vi "Ctor.vi"(8 "error in (no error)":errorcluster, 10 "Role Hierarchy (None)":T1[](array[typedef])) -> (0 "error out":errorcluster, 3 "Security out":refnum<class "Security.lvclass">)   [LabVIEW 2020, in "HTTP Server.lvlib" / "Security.lvclass"]
uses:
  Security.lvclass
  Role Inheritance.ctl
  Ref Data.ctl
  Hierarchy.ctl
  Security.lvclass/Security.ctl
  HTTP Server.lvlib
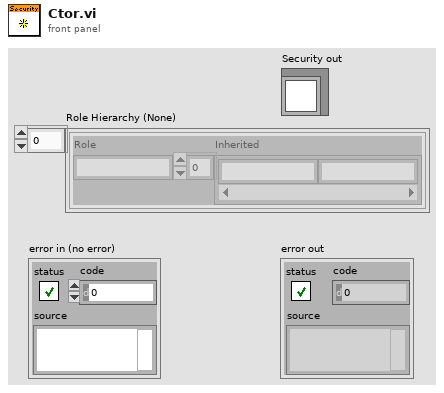
[diagram p1: front panel]
types:
  T1 = typedef "HTTP Server.lvlib/Role Inheritance.ctl" = cluster{"Role":string, "Inherited":string[]}
  T2 = typedef "HTTP Server.lvlib/Security.lvclass/Ref Data.ctl" = cluster{"Hierarchy":T3}
  T3 = typedef "HTTP Server.lvlib/Security.lvclass/Hierarchy.ctl" = map{string, set{string}}
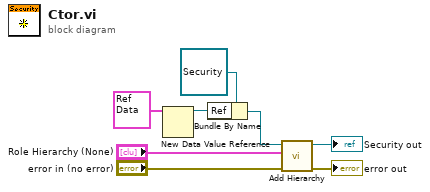
[diagram p0: block diagram]
diagram:
  n1 = New Data Value Reference(data value=T2 {"Hierarchy"={}} ("Ref Data")) -> (data value reference=w6:refnum<data-value>)  [unwired: 1 in, 1 out]
  n2 = Bundle By Name(cluster=refnum<class "Security.lvclass"> refnum ("Security in"), "Ref"=w6) -> (w3:refnum<class "Security.lvclass">)
  n3 = call "Add Hierarchy.vi"("error in (no error)"="error in (no error)", "Hierarchy"="Role Hierarchy (None)", "Security in"=w3) -> ("error out"=→"error out":errorcluster, "Security out"=→"Security out":refnum<class "Security.lvclass">)  [unwired: 7 in]
